vi "eDyno MCU Model.vi"(0 "Speed (rpm)":dbl, 5 "Load Torque (Nm)":dbl, 7 "Motor Parameters":T2={"Kt (Nm per A)"=0.05, "No-load Current (A)"=1.5, "Phase Resistance (ohm)"=0.05, "Iron+Friction Loss (W per rpm)"=0.004, "Battery Voltage (V)"=36.0, "Battery Resistance (ohm)"=0.05, "Ambient Temp (degC)"=25.0, "Winding Rth (K per W)"=0.6, "Controller Rth (K per W)"=0.04}) -> (4 "MCU Status":T1)   [LabVIEW 2026]
doc: "PURPOSE\nSimulates what an e-bike motor controller (MCU) would report on CAN, so the eDyno PoC can log electrical and thermal channels next to vibration. Feeds the MCU_Status frame (0x300) through eDyno CAN Pack Signals.vi. It is a simple STEADY-STATE model for demos - not a validated motor model.\n\nINPUTS\n- Speed (rpm): shaft speed (the simulator's Shaft Speed).\n- Load Torque (Nm): torque at the motor shaft. Positive = motoring, negative = regen. Typical e-bike mid-drive cruise 0.3-1 Nm at the motor shaft (before the gearbox).\n- Motor Parameters: defaults describe a generic 250-500 W, 36 V, 4-pole-pair mid-drive motor. Change them to match a real motor.\n\nOUTPUT (MCU Status cluster, same order as the CAN signals)\nMotor Speed, Torque, Phase Current RMS, DC Voltage, DC Current, Electrical Power, Winding Temp, Controller Temp.\n\nEQUATIONS (one labelled frame each on the block diagram)\n1) omega = rpm x 2pi/60; P_mech = T x omega\n2) I_ph = I_noload + |T|/Kt; P_copper = 3 x R_ph x I_ph^2; P_iron+friction = k x rpm; P_loss = sum\n3) P_elec = P_mech + P_loss; V_dc = V_batt - R_batt x P_elec/V_batt; I_dc = P_elec/V_dc\n4) T_winding = T_amb + Rth_w x P_loss; T_controller = T_amb + Rth_c x |P_elec|\n\nEXAMPLE (defaults): 4500 rpm, 0.5 Nm -> 11.5 A rms, 273 W, 35.6 V, 7.7 A DC, winding 47.7 degC, controller 35.9 degC.\n\nLIMITATIONS\nTemperatures jump instantly (no thermal time constant); efficiency map is approximate; field weakening, voltage limit and current limit are not modelled."
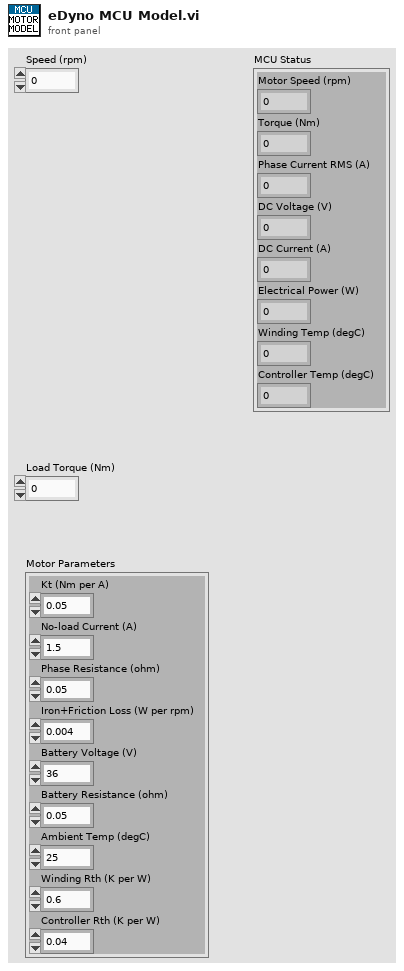
[diagram p1: front panel]
types:
  T1 = cluster{"Motor Speed (rpm)":dbl, "Torque (Nm)":dbl, "Phase Current RMS (A)":dbl, "DC Voltage (V)":dbl, "DC Current (A)":dbl, "Electrical Power (W)":dbl, "Winding Temp (degC)":dbl, "Controller Temp (degC)":dbl}
  T2 = cluster{"Kt (Nm per A)":dbl, "No-load Current (A)":dbl, "Phase Resistance (ohm)":dbl, "Iron+Friction Loss (W per rpm)":dbl, "Battery Voltage (V)":dbl, "Battery Resistance (ohm)":dbl, "Ambient Temp (degC)":dbl, "Winding Rth (K per W)":dbl, "Controller Rth (K per W)":dbl}
  T3 = cluster{"Speed (rpm)":dbl, "Load Torque (Nm)":dbl, dbl, dbl, dbl, dbl, dbl, dbl}
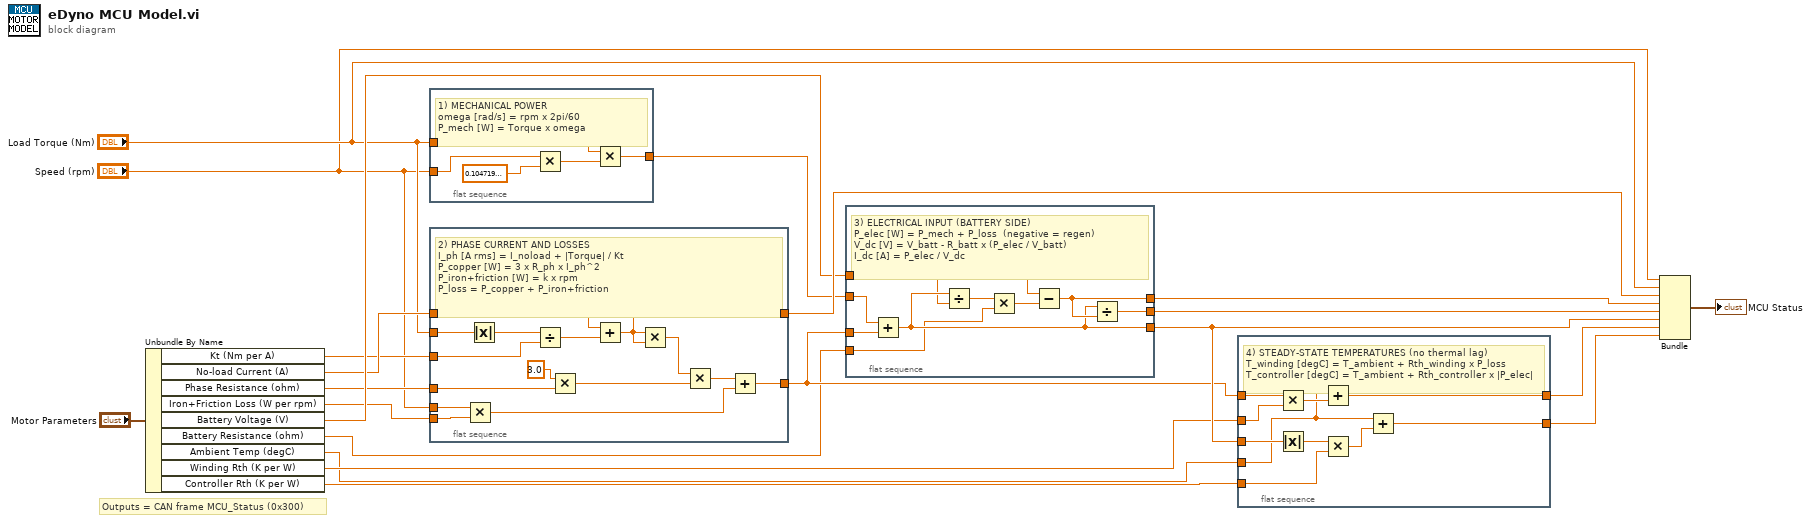
[diagram p0: block diagram]
diagram:
  # "Outputs = CAN frame MCU_Status (0x300)"
  n1 = Unbundle By Name("Motor Parameters") -> ("Kt (Nm per A)"=w4:dbl, "No-load Current (A)"=w5:dbl, "Phase Resistance (ohm)"=w6:dbl, "Iron+Friction Loss (W per rpm)"=w7:dbl, "Battery Voltage (V)"=w8:dbl, "Battery Resistance (ohm)"=w9:dbl, "Ambient Temp (degC)"=w10:dbl, "Winding Rth (K per W)"=w11:dbl, "Controller Rth (K per W)"=w12:dbl)
  n2 = flat-sequence {
    tunnel: "Speed (rpm)" -> [w22]
    tunnel: "Load Torque (Nm)" -> [w23]
    tunnel: [w26] -> w13
    frame #0 {
      # "1) MECHANICAL POWER\nomega [rad/s] = rpm x 2pi/60\nP_mech [W] = Torque x omega"
      n3 = Multiply(x=w22, y=0.10471975511965977 ("2pi/60 (rad/s per rpm)")) -> (x*y=w25:dbl)
      n4 = Multiply(x=w23, y=w25) -> (x*y=w26:dbl)
    }
  }
  n5 = flat-sequence {
    tunnel: "Load Torque (Nm)" -> [w28]
    tunnel: "Speed (rpm)" -> [w31]
    tunnel: w5 -> [w27]
    tunnel: w4 -> [w29]
    tunnel: w6 -> [w30]
    tunnel: w7 -> [w32]
    tunnel: [w35] -> w14
    tunnel: [w41] -> w15
    frame #0 {
      # "2) PHASE CURRENT AND LOSSES\nI_ph [A rms] = I_noload + |Torque| / Kt\nP_copper [W] = 3 x R_ph x I_ph^2\nP_iron+friction [W] = k x rpm\nP_loss = P_copper + P_iron+friction"
      n6 = Multiply(x=w31, y=w32) -> (x*y=w40:dbl)
      n7 = Absolute Value(x=w28) -> (abs(x)=w33:dbl)
      n8 = Divide(x=w33, y=w29) -> (x/y=w34:dbl)
      n9 = Multiply(x=3.0 ("3 phases"), y=w30) -> (x*y=w38:dbl)
      n10 = Add(x=w27, y=w34) -> (x+y=w35:dbl)
      n11 = Multiply(x=w35, y=w35) -> (x*y=w36:dbl)
      n12 = Multiply(x=w36, y=w38) -> (x*y=w39:dbl)
      n13 = Add(x=w39, y=w40) -> (x+y=w41:dbl)
    }
  }
  n14 = flat-sequence {
    tunnel: w8 -> [w44]
    tunnel: w9 -> [w45]
    tunnel: w13 -> [w42]
    tunnel: w15 -> [w43]
    tunnel: [w46] -> w16
    tunnel: [w49] -> w17
    tunnel: [w50] -> w18
    frame #0 {
      # "3) ELECTRICAL INPUT (BATTERY SIDE)\nP_elec [W] = P_mech + P_loss  (negative = regen)\nV_dc [V] = V_batt - R_batt x (P_elec / V_batt)\nI_dc [A] = P_elec / V_dc"
      n15 = Add(x=w42, y=w43) -> (x+y=w46:dbl)
      n16 = Divide(x=w46, y=w44) -> (x/y=w47:dbl)
      n17 = Multiply(x=w47, y=w45) -> (x*y=w48:dbl)
      n18 = Subtract(x=w44, y=w48) -> (x-y=w49:dbl)
      n19 = Divide(x=w46, y=w49) -> (x/y=w50:dbl)
    }
  }
  n20 = flat-sequence {
    tunnel: w10 -> [w51]
    tunnel: w11 -> [w53]
    tunnel: w12 -> [w55]
    tunnel: w15 -> [w52]
    tunnel: w16 -> [w54]
    tunnel: [w57] -> w19
    tunnel: [w60] -> w20
    frame #0 {
      # "4) STEADY-STATE TEMPERATURES (no thermal lag)\nT_winding [degC] = T_ambient + Rth_winding x P_loss\nT_controller [degC] = T_ambient + Rth_controller x |P_elec|"
      n21 = Multiply(x=w52, y=w53) -> (x*y=w56:dbl)
      n22 = Absolute Value(x=w54) -> (abs(x)=w58:dbl)
      n23 = Add(x=w51, y=w56) -> (x+y=w57:dbl)
      n24 = Multiply(x=w58, y=w55) -> (x*y=w59:dbl)
      n25 = Add(x=w51, y=w59) -> (x+y=w60:dbl)
    }
  }
  n26 = Bundle("Speed (rpm)"="Speed (rpm)", "Load Torque (Nm)"="Load Torque (Nm)", w14, w17, w18, w16, w19, w20) -> (→"MCU Status":T3)  [unwired: 1 in]
